vi "Mock Circulation Loop met sub-Vi - AANGEPAST VOOR CHARLOTTE.vi"() -> ()   [LabVIEW 2024]
uses:
  <vilib>/DAQmx/write.llb/DAQmx Write (Analog DBL 1Chan 1Samp).vi
  <vilib>/DAQmx/read.llb/DAQmx Read (Analog 1D DBL NChan 1Samp).vi
  <vilib>/DAQmx/write.llb/DAQmx Write (Digital 1D Bool NChan 1Samp 1Line).vi
  <vilib>/DAQmx/create/channels.llb/DAQmx Create Channel (DO-Digital Output).vi
  <vilib>/DAQmx/miscellaneous.llb/DAQmx Fill In Error Info.vi
  <vilib>/DAQmx/create/channels.llb/DAQmx Create Channel (AI-Voltage-Basic).vi
  <vilib>/DAQmx/create/channels.llb/DAQmx Create Channel (AO-Voltage-Basic).vi
  <vilib>/Utility/file.llb/Write Delimited Spreadsheet (string).vi
  <vilib>/Utility/file.llb/Write Delimited Spreadsheet (DBL).vi
panel:
  in  "Set pressure Hybrid Heart (Bar)":dbl
  in  "Analog output pressure regulator":tag="Dev1/ao0"
  out "Actual Press. from Regulator (Bar)":dbl=0.5073311185231432
  out "Flow sensors":cluster{dbl[], dbl[]}[](graph)=[{[0.014721000000463391], [-6.750071131370961, -6.750071131370961, -6.750071131370961, -6.750071131370961, -6.750071131370961, -6.750071131370961, -6.750071131370961, -6.750071131370961, -6.750071131370961, -6.750071131370961, -6.750071131370961, -6.750071131370961, -6.750071131370961, -6.750071131370961, -6.750071131370961, -6.750071131370961, -6.755156296628295, -6.755156296628295, -6.750071131370961, -6.750071131370961, -6.750071131370961, -6.750071131370961, -6.750071131370961, -6.750071131370961, -6.750071131370961, -6.750071131370961, -6.750071131370961, -6.755156296628295, -6.750071131370961, -6.750071131370961, -6.750071131370961, -6.750071131370961, -6.750071131370961, -6.750071131370961, -6.750071131370961, -6.750071131370961, -6.750071131370961, -6.750071131370961, -6.750071131370961, -6.750071131370961, -6.750071131370961, -6.750071131370961, -6.750071131370961, -6.750071131370961, -6.750071131370961, -6.750071131370961, -6.750071131370961, -6.750071131370961, -6.750071131370961, -6.750071131370961, -6.750071131370961, -6.750071131370961, -6.750071131370961, -6.750071131370961, -6.750071131370961, -6.750071131370961, -6.750071131370961, -6.750071131370961, -6.750071131370961, -6.750071131370961, -6.750071131370961, -6.750071131370961, -6.750071131370961, -6.750071131370961, -6.750071131370961, -6.750071131370961, -6.750071131370961, -6.750071131370961, -6.750071131370961, -6.750071131370961, -6.755156296628295, -6.750071131370961, -6.750071131370961, -6.750071131370961, -6.750071131370961, -6.750071131370961, -6.755156296628295, -6.750071131370961, -6.750071131370961, -6.750071131370961, -6.750071131370961, -6.750071131370961, -6.750071131370961, -6.750071131370961, -6.750071131370961, -6.750071131370961, -6.750071131370961, -6.750071131370961, -6.750071131370961, -6.750071131370961, -6.750071131370961, -6.750071131370961, -6.750071131370961, -6.755156296628295, -6.744985966113629, -6.750071131370961, -6.750071131370961, -6.750071131370961, -6.750071131370961, -6.750071131370961, -6.750071131370961, -6.750071131370961, -6.750071131370961, -6.750071131370961, -6.750071131370961, -6.750071131370961, -6.750071131370961, -6.750071131370961, -6.755156296628295, -6.750071131370961, -6.750071131370961, -6.750071131370961, -6.750071131370961, -6.755156296628295, -6.750071131370961, -6.750071131370961, -6.750071131370961, -6.750071131370961, -6.750071131370961, -6.750071131370961, -6.755156296628295, -6.750071131370961, -6.750071131370961, -6.750071131370961, -6.750071131370961, -6.750071131370961, -6.750071131370961, -6.750071131370961, -6.750071131370961, -6.750071131370961, -6.750071131370961, -6.755156296628295, -6.750071131370961, -6.750071131370961, -6.750071131370961, -6.750071131370961, -6.750071131370961, -6.750071131370961, -6.750071131370961, -6.750071131370961, -6.750071131370961, -6.750071131370961, -6.750071131370961, -6.750071131370961, -6.750071131370961, -6.750071131370961, -6.755156296628295, -6.750071131370961, -6.750071131370961, -6.750071131370961, -6.750071131370961, -6.750071131370961, -6.750071131370961, -6.750071131370961, -6.750071131370961, -6.750071131370961, -6.750071131370961, -6.750071131370961, -6.750071131370961, -6.750071131370961, -6.750071131370961, -6.750071131370961, -6.750071131370961, -6.750071131370961, -6.750071131370961, -6.750071131370961, -6.750071131370961, -6.750071131370961, -6.744985966113629, -6.750071131370961, -6.750071131370961, -6.750071131370961, -6.750071131370961, -6.750071131370961, -6.750071131370961, -6.750071131370961, -6.750071131370961, -6.750071131370961, -6.750071131370961, -6.750071131370961, -6.750071131370961, -6.750071131370961, -6.750071131370961, -6.750071131370961, -6.750071131370961, -6.750071131370961, -6.750071131370961, -6.750071131370961, -6.750071131370961, -6.755156296628295, -6.755156296628295, -6.750071131370961, -6.750071131370961, -6.750071131370961, -6.750071131370961, -6.750071131370961, -6.750071131370961, -6.750071131370961, -6.744985966113629, -6.750071131370961, -6.750071131370961, -6.750071131370961, -6.750071131370961, -6.750071131370961, -6.750071131370961, -6.750071131370961, -6.750071131370961, -6.750071131370961, -6.750071131370961, -6.750071131370961, -6.750071131370961, -6.750071131370961, -6.750071131370961, -6.755156296628295, -6.750071131370961, -6.750071131370961, -6.750071131370961, -6.750071131370961, -6.750071131370961, -6.755156296628295, -6.750071131370961, -6.750071131370961, -6.750071131370961, -6.750071131370961, -6.750071131370961, -6.750071131370961, -6.750071131370961, -6.750071131370961, -6.750071131370961, -6.750071131370961, -6.750071131370961, -6.750071131370961, -6.750071131370961, -6.750071131370961, -6.750071131370961, -6.750071131370961, -6.750071131370961, -6.750071131370961, -6.750071131370961, -6.750071131370961, -6.750071131370961, -6.750071131370961, -6.750071131370961, -6.750071131370961, -6.750071131370961, -6.750071131370961, -6.750071131370961, -6.750071131370961, -6.750071131370961, -6.750071131370961, -6.750071131370961, -6.750071131370961, -6.750071131370961, -6.755156296628295, -6.750071131370961, -6.750071131370961, -6.750071131370961, -6.755156296628295, -6.750071131370961, -6.750071131370961, -6.750071131370961, -6.750071131370961, -6.750071131370961, -6.750071131370961, -6.755156296628295, -6.750071131370961, -6.750071131370961, -6.750071131370961, -6.750071131370961, -6.750071131370961, -6.750071131370961, -6.750071131370961, -6.750071131370961, -6.750071131370961, -6.750071131370961, -6.750071131370961, -6.750071131370961, -6.750071131370961, -6.750071131370961, -6.750071131370961, -6.750071131370961, -6.750071131370961, -6.750071131370961, -6.750071131370961, -6.750071131370961, -6.750071131370961, -6.750071131370961, -6.750071131370961, -6.750071131370961, -6.750071131370961, -6.755156296628295, -6.750071131370961, -6.750071131370961, -6.750071131370961, -6.750071131370961, -6.750071131370961, -6.750071131370961, -6.750071131370961, -6.750071131370961, -6.755156296628295, -6.750071131370961, -6.750071131370961, -6.750071131370961, -6.750071131370961, -6.755156296628295, -6.750071131370961, -6.755156296628295, -6.750071131370961, -6.750071131370961, -6.750071131370961, -6.750071131370961, -6.750071131370961, -6.750071131370961, -6.750071131370961, -6.750071131370961, -6.750071131370961, -6.750071131370961, -6.750071131370961, -6.750071131370961, -6.750071131370961, -6.750071131370961, -6.750071131370961, -6.750071131370961, -6.750071131370961, -6.750071131370961, -6.750071131370961, -6.750071131370961, -6.750071131370961, -6.750071131370961, -6.750071131370961, -6.750071131370961, -6.750071131370961, -6.750071131370961, -6.750071131370961, -6.750071131370961, -6.750071131370961, -6.750071131370961, -6.750071131370961, -6.750071131370961, -6.750071131370961, -6.750071131370961, -6.750071131370961, -6.750071131370961, -6.750071131370961, -6.750071131370961, -6.750071131370961, -6.755156296628295, -6.750071131370961, -6.750071131370961, -6.750071131370961, -6.750071131370961, -6.750071131370961, -6.750071131370961, -6.750071131370961, -6.750071131370961, -6.750071131370961, -6.755156296628295, -6.750071131370961, -6.750071131370961, -6.750071131370961, -6.750071131370961, -6.750071131370961, -6.750071131370961, -6.750071131370961, -6.750071131370961, -6.750071131370961, -6.750071131370961, -6.750071131370961, -6.750071131370961, -6.750071131370961, -6.750071131370961, -6.750071131370961, -6.750071131370961, -6.750071131370961, -6.750071131370961, -6.750071131370961, -6.750071131370961, -6.750071131370961, -6.750071131370961, -6.750071131370961, -6.750071131370961, -6.750071131370961, -6.750071131370961, -6.750071131370961, -6.750071131370961, -6.750071131370961, -6.750071131370961, -6.744985966113629, -6.750071131370961, -6.750071131370961, -6.750071131370961, -6.750071131370961, -6.750071131370961, -6.750071131370961, -6.750071131370961, -6.755156296628295, -6.750071131370961, -6.750071131370961, -6.750071131370961, -6.750071131370961, -6.750071131370961, -6.750071131370961, -6.750071131370961, -6.755156296628295, -6.750071131370961]}, ...(2 in all)]
  in  "Seconds per data point":dbl
  out "Pressure sensors":cluster{dbl[], dbl[]}[](graph)=[{[0.014721000000463391], [-2.2408081975299865, -2.2408081975299865, -2.4339157389476895, -2.2408081975299865, -1.8545931146945804, -2.4339157389476895, -2.2408081975299865, -2.2408081975299865, -2.2408081975299865, -2.2408081975299865, -2.4339157389476895, -2.4339157389476895, -2.4339157389476895, -2.4339157389476895, -2.4339157389476895, -2.2408081975299865, -2.2408081975299865, -2.2408081975299865, -2.4339157389476895, -2.2408081975299865, -2.4339157389476895, -2.2408081975299865, -2.4339157389476895, -2.2408081975299865, -2.2408081975299865, -2.2408081975299865, -2.2408081975299865, -2.2408081975299865, -2.4339157389476895, -2.2408081975299865, -2.4339157389476895, -2.2408081975299865, -2.4339157389476895, -2.4339157389476895, -2.4339157389476895, -2.4339157389476895, -2.4339157389476895, -2.2408081975299865, -2.2408081975299865, -2.2408081975299865, -2.4339157389476895, -2.2408081975299865, -2.4339157389476895, -2.4339157389476895, -2.4339157389476895, -2.2408081975299865, -2.2408081975299865, -2.2408081975299865, -2.4339157389476895, -2.2408081975299865, -2.4339157389476895, -2.4339157389476895, -2.2408081975299865, -2.2408081975299865, -2.4339157389476895, -2.4339157389476895, -2.2408081975299865, -2.2408081975299865, -2.2408081975299865, -2.4339157389476895, -2.4339157389476895, -2.2408081975299865, -2.4339157389476895, -2.4339157389476895, -2.4339157389476895, -2.4339157389476895, -2.4339157389476895, -2.4339157389476895, -2.2408081975299865, -2.2408081975299865, -2.2408081975299865, -2.4339157389476895, -2.2408081975299865, -2.4339157389476895, -2.2408081975299865, -2.2408081975299865, -2.4339157389476895, -2.4339157389476895, -2.4339157389476895, -2.4339157389476895, -2.4339157389476895, -2.4339157389476895, -2.4339157389476895, -2.4339157389476895, -2.4339157389476895, -2.4339157389476895, -2.4339157389476895, -2.2408081975299865, -2.4339157389476895, -2.4339157389476895, -2.2408081975299865, -2.4339157389476895, -2.4339157389476895, -2.2408081975299865, -2.4339157389476895, -2.4339157389476895, -2.4339157389476895, -2.2408081975299865, -2.4339157389476895, -2.4339157389476895, -2.4339157389476895, -2.2408081975299865, -2.4339157389476895, -2.4339157389476895, -2.2408081975299865, -2.2408081975299865, -2.4339157389476895, -2.4339157389476895, -2.2408081975299865, -2.4339157389476895, -2.4339157389476895, -2.0477006561122835, -2.4339157389476895, -2.2408081975299865, -2.4339157389476895, -2.2408081975299865, -2.2408081975299865, -2.4339157389476895, -2.0477006561122835, -2.2408081975299865, -2.2408081975299865, -2.4339157389476895, -2.2408081975299865, -2.4339157389476895, -2.4339157389476895, -2.4339157389476895, -2.4339157389476895, -2.4339157389476895, -2.2408081975299865, -2.0477006561122835, -2.4339157389476895, -2.4339157389476895, -2.4339157389476895, -2.2408081975299865, -2.4339157389476895, -2.4339157389476895, -2.4339157389476895, -2.4339157389476895, -2.2408081975299865, -2.4339157389476895, -2.4339157389476895, -2.4339157389476895, -2.2408081975299865, -2.4339157389476895, -2.4339157389476895, -2.4339157389476895, -2.4339157389476895, -2.4339157389476895, -2.2408081975299865, -2.4339157389476895, -2.4339157389476895, -1.8545931146945804, -2.2408081975299865, -2.4339157389476895, -2.2408081975299865, -2.2408081975299865, -2.4339157389476895, -2.2408081975299865, -2.4339157389476895, -2.0477006561122835, -2.4339157389476895, -2.2408081975299865, -2.0477006561122835, -2.4339157389476895, -2.4339157389476895, -2.2408081975299865, -2.2408081975299865, -2.4339157389476895, -2.2408081975299865, -2.4339157389476895, -2.2408081975299865, -2.4339157389476895, -2.2408081975299865, -2.2408081975299865, -2.4339157389476895, -2.4339157389476895, -2.4339157389476895, -2.0477006561122835, -2.2408081975299865, -2.4339157389476895, -2.2408081975299865, -2.4339157389476895, -2.2408081975299865, -2.4339157389476895, -2.4339157389476895, -2.4339157389476895, -2.4339157389476895, -2.2408081975299865, -2.4339157389476895, -2.4339157389476895, -2.2408081975299865, -2.2408081975299865, -2.4339157389476895, -2.4339157389476895, -2.2408081975299865, -2.4339157389476895, -2.4339157389476895, -2.2408081975299865, -2.2408081975299865, -2.4339157389476895, -2.4339157389476895, -2.2408081975299865, -2.2408081975299865, -2.2408081975299865, -2.2408081975299865, -2.2408081975299865, -2.4339157389476895, -2.4339157389476895, -2.4339157389476895, -2.2408081975299865, -2.4339157389476895, -2.2408081975299865, -2.4339157389476895, -2.6270232803653926, -2.4339157389476895, -2.2408081975299865, -2.2408081975299865, -2.2408081975299865, -2.4339157389476895, -2.4339157389476895, -2.2408081975299865, -2.4339157389476895, -2.4339157389476895, -2.2408081975299865, -2.4339157389476895, -2.4339157389476895, -2.4339157389476895, -2.2408081975299865, -2.4339157389476895, -1.8545931146945804, -2.4339157389476895, -2.4339157389476895, -2.4339157389476895, -2.4339157389476895, -2.4339157389476895, -2.0477006561122835, -2.4339157389476895, -2.4339157389476895, -2.2408081975299865, -2.4339157389476895, -2.2408081975299865, -2.4339157389476895, -2.4339157389476895, -2.4339157389476895, -2.2408081975299865, -2.2408081975299865, -1.8545931146945804, -2.4339157389476895, -2.4339157389476895, -2.2408081975299865, -2.4339157389476895, -2.4339157389476895, -2.4339157389476895, -2.4339157389476895, -2.4339157389476895, -2.4339157389476895, -2.4339157389476895, -2.2408081975299865, -2.2408081975299865, -2.4339157389476895, -2.4339157389476895, -2.4339157389476895, -2.2408081975299865, -2.4339157389476895, -2.4339157389476895, -2.4339157389476895, -2.4339157389476895, -2.4339157389476895, -2.4339157389476895, -2.4339157389476895, -2.4339157389476895, -2.4339157389476895, -2.4339157389476895, -2.2408081975299865, -2.4339157389476895, -2.4339157389476895, -2.2408081975299865, -2.4339157389476895, -2.2408081975299865, -2.2408081975299865, -2.4339157389476895, -2.4339157389476895, -2.2408081975299865, -2.4339157389476895, -2.4339157389476895, -2.4339157389476895, -2.2408081975299865, -2.4339157389476895, -2.2408081975299865, -2.4339157389476895, -2.2408081975299865, -2.4339157389476895, -2.4339157389476895, -2.2408081975299865, -2.2408081975299865, -2.4339157389476895, -2.4339157389476895, -1.8545931146945804, -2.4339157389476895, -2.2408081975299865, -2.2408081975299865, -2.4339157389476895, -2.4339157389476895, -2.2408081975299865, -2.4339157389476895, -2.2408081975299865, -2.4339157389476895, -2.2408081975299865, -2.4339157389476895, -2.2408081975299865, -2.2408081975299865, -2.2408081975299865, -2.2408081975299865, -2.2408081975299865, -2.2408081975299865, -2.4339157389476895, -2.2408081975299865, -2.4339157389476895, -2.4339157389476895, -2.4339157389476895, -2.2408081975299865, -2.4339157389476895, -2.4339157389476895, -2.4339157389476895, -2.2408081975299865, -2.2408081975299865, -2.2408081975299865, -2.4339157389476895, -2.2408081975299865, -2.4339157389476895, -2.4339157389476895, -2.4339157389476895, -2.2408081975299865, -2.4339157389476895, -2.4339157389476895, -2.2408081975299865, -2.4339157389476895, -2.4339157389476895, -2.4339157389476895, -2.2408081975299865, -2.4339157389476895, -2.4339157389476895, -2.2408081975299865, -2.4339157389476895, -2.0477006561122835, -2.4339157389476895, -2.4339157389476895, -2.4339157389476895, -2.2408081975299865, -2.4339157389476895, -2.4339157389476895, -2.2408081975299865, -2.4339157389476895, -2.4339157389476895, -2.2408081975299865, -2.4339157389476895, -2.2408081975299865, -2.4339157389476895, -2.4339157389476895, -2.4339157389476895, -2.2408081975299865, -2.4339157389476895, -2.4339157389476895, -2.4339157389476895, -2.2408081975299865, -2.4339157389476895, -2.4339157389476895, -2.4339157389476895, -2.2408081975299865, -2.4339157389476895, -2.2408081975299865, -2.4339157389476895, -2.4339157389476895, -2.4339157389476895, -2.2408081975299865, -1.8545931146945804, -2.4339157389476895, -2.2408081975299865, -2.4339157389476895, -2.4339157389476895, -2.2408081975299865, -2.2408081975299865, -2.4339157389476895, -2.2408081975299865, -2.4339157389476895, -2.4339157389476895, -2.2408081975299865, -2.4339157389476895, -2.2408081975299865, -2.2408081975299865, -2.4339157389476895, -2.2408081975299865, -2.2408081975299865, -2.2408081975299865, -2.4339157389476895, -2.4339157389476895, -2.4339157389476895, -2.4339157389476895, -2.2408081975299865, -2.4339157389476895, -2.2408081975299865, -2.4339157389476895, -2.4339157389476895, -2.2408081975299865, -2.2408081975299865]}, ...(2 in all)]
  out "Elapsed time":dbl=0.014721000000463391
  in  "Input port all sensors":tag="Dev1/ai3:7"
  in  "Start/Stop solenoid valves":bool
  in  "Closed time (ms)":dbl=700.0
  in  "Open time (ms)":dbl=300.0
  in  "STOP":bool
  in  "line grouping":i32(ring) items=["one channel for each line", "one channel for all lines"]
  in  "Port input Solenoid valve":tag="Dev1/port0/line0:1"
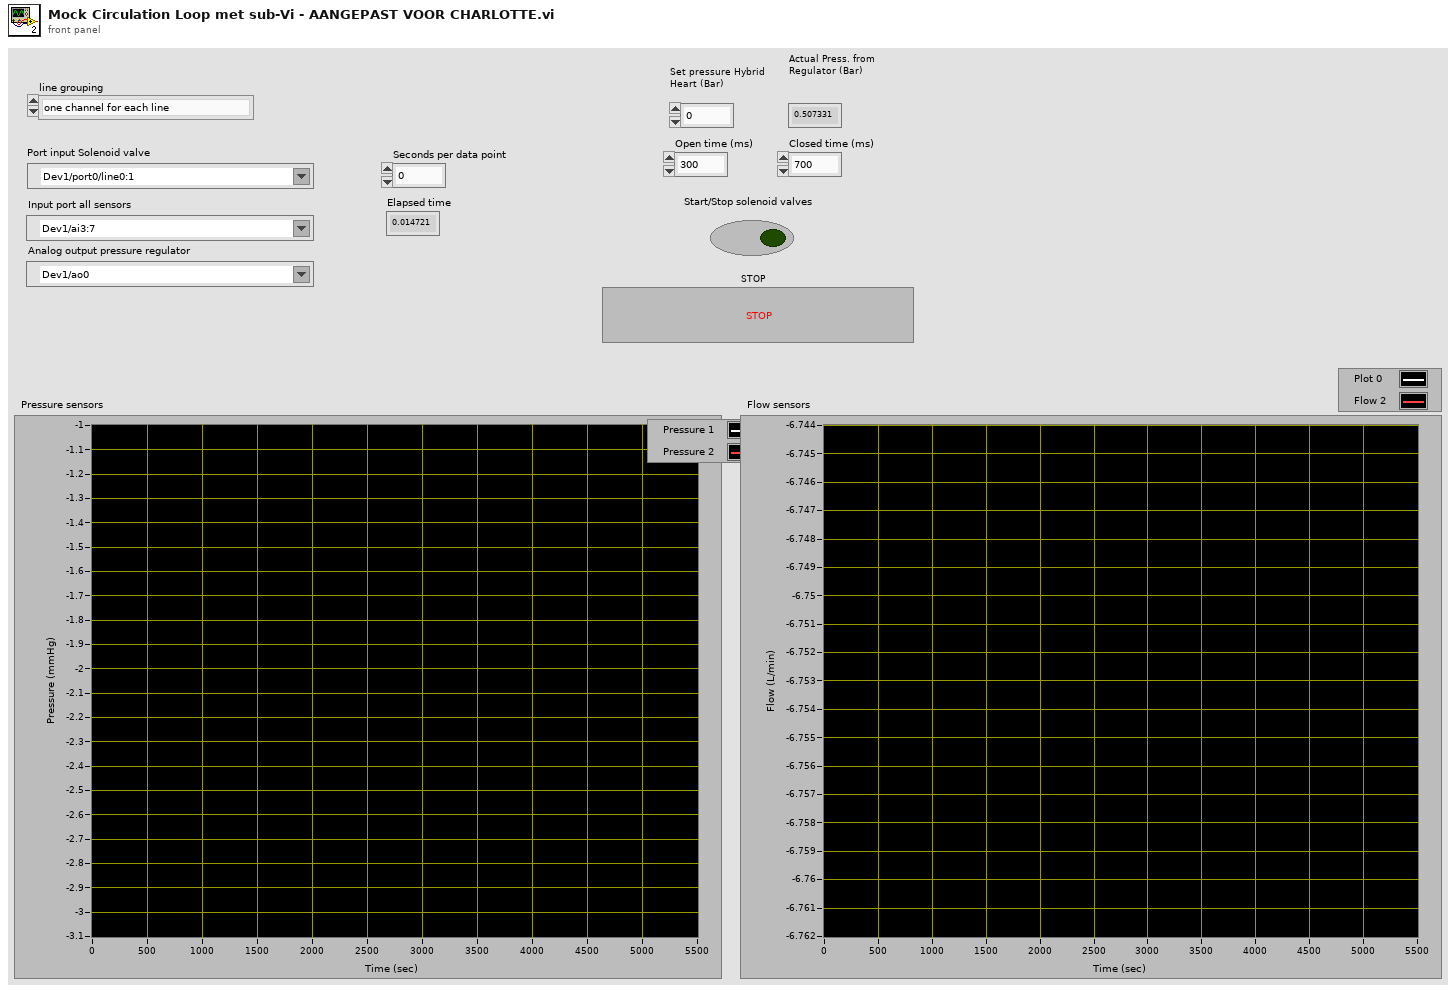
[diagram p1: front panel]
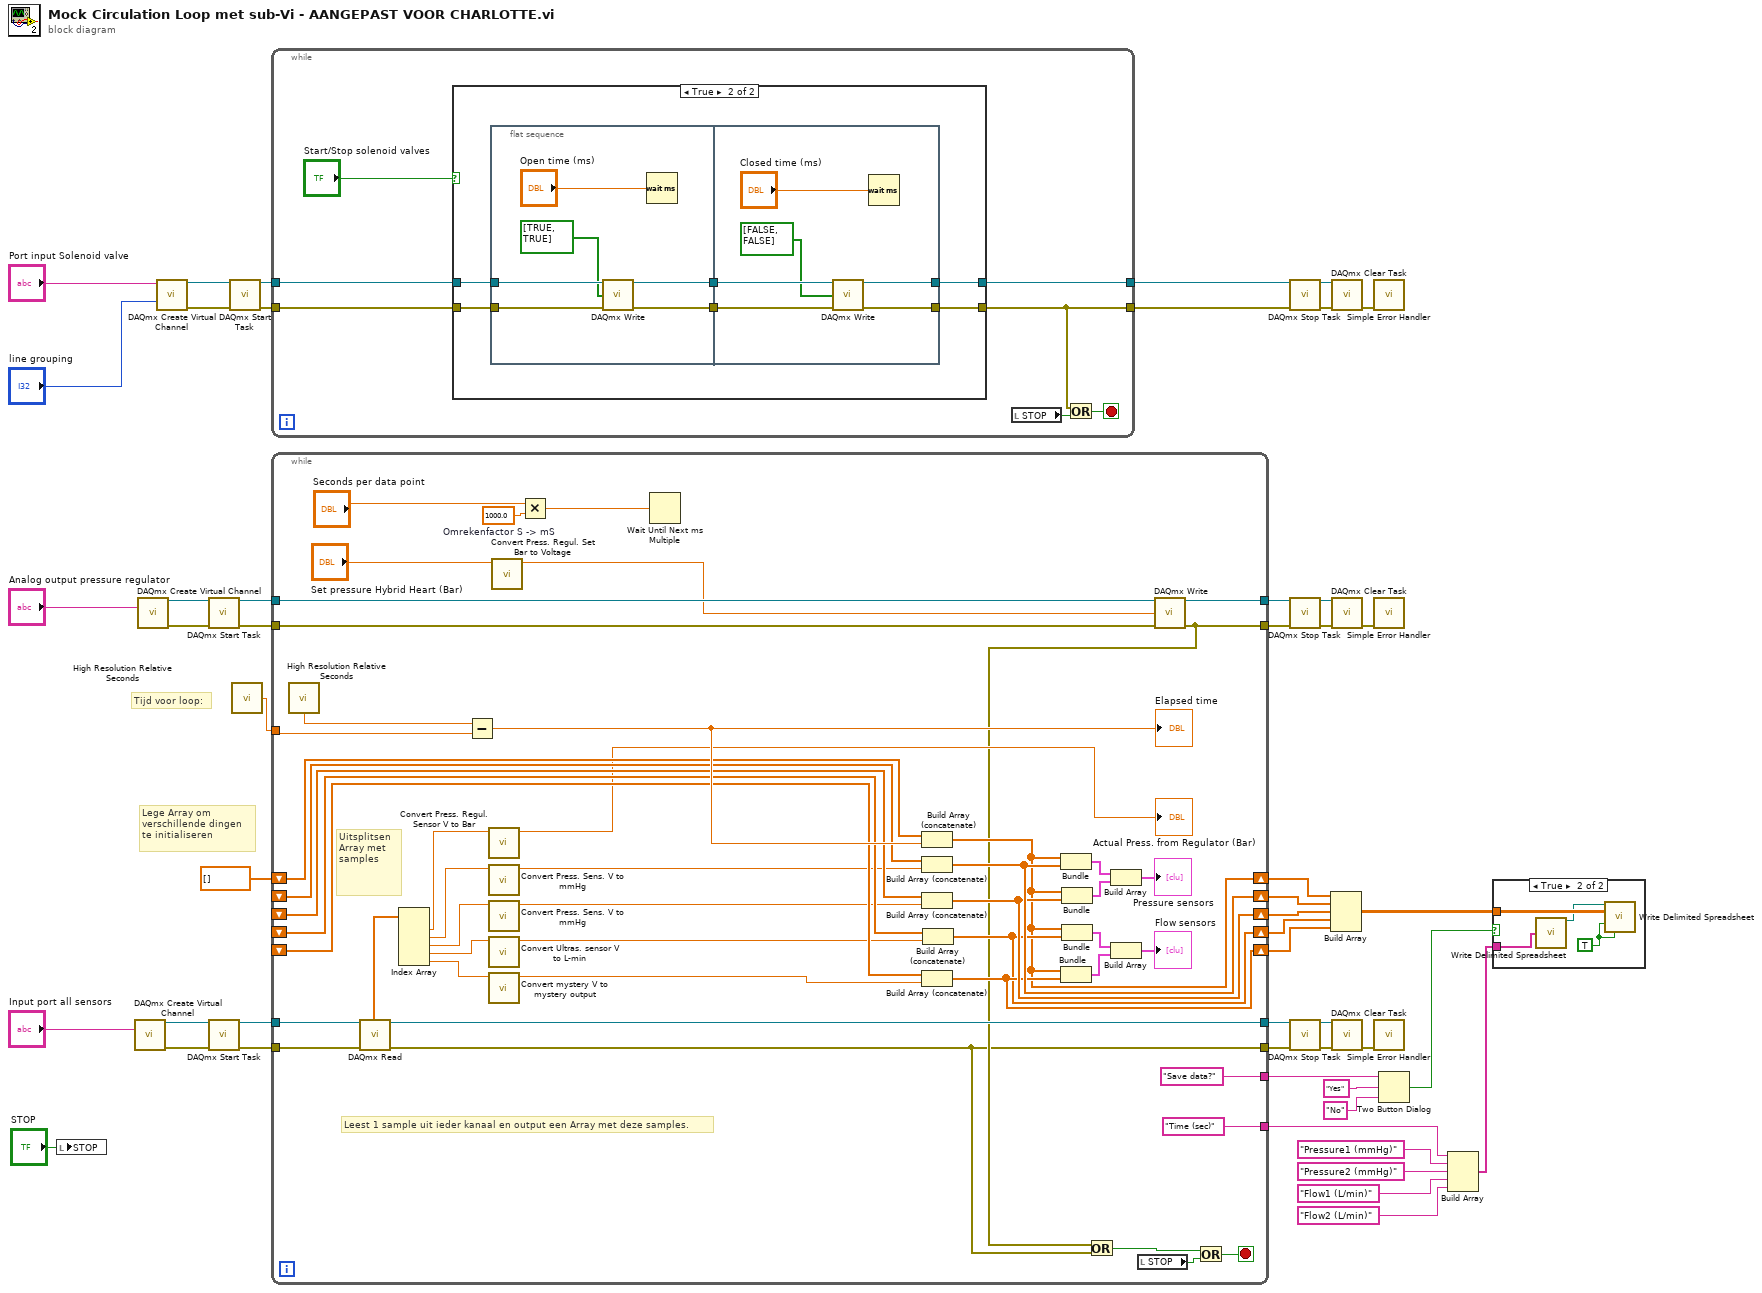
[diagram p0: block diagram]
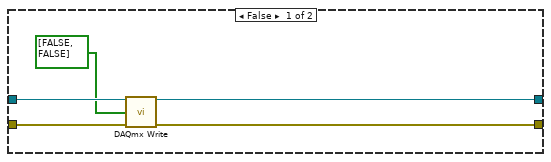
[diagram p3: hidden frame]
diagram:
  # "Tijd voor loop:"
  # "Lege Array om\nverschillende dingen \nte initialiseren"
  n1 = local write "STOP"("STOP") -> ()
  n2 = call-poly <vilib>:"DAQmx Create Virtual Channel.vi"("physical channels"="Input port all sensors") -> ("task out"=w36:refnum<k21>, "error out"=w35:errorcluster)  [unwired: 13 in]
  n3 = call-poly <vilib>:"DAQmx Create Virtual Channel.vi"("physical channels"="Analog output pressure regulator") -> ("task out"=w27:refnum<k21>, "error out"=w26:errorcluster)  [unwired: 13 in]
  n4 = call-poly <vilib>:"DAQmx Create Virtual Channel.vi"("lines"="Port input Solenoid valve", "line grouping"="line grouping") -> ("task out"=w48:refnum<k21>, "error out"=w49:errorcluster)  [unwired: 12 in]
  n5 = call <vilib>:"DAQmx Start Task.vi"("task/channels in"=w27, "error in"=w26) -> ("task out"=w23:refnum<k21>, "error out"=w24:errorcluster)  [unwired: 12 in]
  n6 = call <vilib>:"DAQmx Start Task.vi"("task/channels in"=w36, "error in"=w35) -> ("task out"=w34:refnum<k21>, "error out"=w33:errorcluster)  [unwired: 12 in]
  n7 = call <vilib>:"DAQmx Start Task.vi"("task/channels in"=w48, "error in"=w49) -> ("task out"=w46:refnum<k21>, "error out"=w45:errorcluster)  [unwired: 12 in]
  n8 = call <vilib>:"High Resolution Relative Seconds.vi"() -> ("relative seconds"=w38:dbl)
  n9 = while {
    tunnel: w46 -> [w56]
    tunnel: w45 -> [w55]
    tunnel: [w52] -> w43
    tunnel: [w54] -> w42
    stop <- w53 stop-if-true
    n10 = case shown="True" "Start/Stop solenoid valves" {
      tunnel: w56 -> [w62 w66]
      tunnel: w55 -> [w61 w65]
      tunnel: [w59 w64] -> w52
      tunnel: [w58 w63] -> w54
      frame False {
        n11 = call-poly <vilib>:"DAQmx Write.vi"("task/channels in"=w62, "data"=bool[] [FALSE, FALSE], "error in"=w61) -> ("task out"=w58:refnum<k21>, "error out"=w59:errorcluster)  [unwired: 10 in, 1 out]
      }
      frame True {
        n12 = flat-sequence {
          tunnel: w66 -> [w74]
          tunnel: w65 -> [w73]
          tunnel: [w71] -> w68
          tunnel: [w70] -> w67
          tunnel: w68 -> [w79]
          tunnel: w67 -> [w78]
          tunnel: [w77] -> w63
          tunnel: [w76] -> w64
          frame #0 {
            n13 = call-poly <vilib>:"DAQmx Write.vi"("task/channels in"=w74, "data"=bool[] [TRUE, TRUE], "error in"=w73) -> ("task out"=w71:refnum<k21>, "error out"=w70:errorcluster)  [unwired: 10 in, 1 out]
            n14 = Wait (ms)(milliseconds to wait="Open time (ms)") -> ()  [unwired: 1 out]
          }
          frame #1 {
            n15 = call-poly <vilib>:"DAQmx Write.vi"("task/channels in"=w79, "data"=bool[] [FALSE, FALSE], "error in"=w78) -> ("task out"=w77:refnum<k21>, "error out"=w76:errorcluster)  [unwired: 10 in, 1 out]
            n16 = Wait (ms)(milliseconds to wait="Closed time (ms)") -> ()  [unwired: 1 out]
          }
        }
      }
    }
    n17 = local read "STOP"() -> (w51:bool)
    n18 = Or(x=w52, y=w51) -> (x .or. y?=w53:bool)
  }
  n19 = while {
    tunnel: w34 -> [w128]
    tunnel: w33 -> [w127]
    tunnel: w38 -> [w122]
    shift-right: [w106] -> w17
    shift-left: dbl[] [] -> [w120]
    shift-right: [w116] -> w16
    shift-left: _ -> [w118]
    shift-right: [w115] -> w15
    shift-left: _ -> [w117]
    tunnel: [w111] -> w32
    tunnel: [w82] -> w31
    shift-right: [w107] -> w14
    shift-left: _ -> [w110]
    shift-right: [w108] -> w13
    shift-left: _ -> [w109]
    tunnel: w24 -> [w81]
    tunnel: w23 -> [w102]
    tunnel: [w83] -> w19
    tunnel: [w101] -> w18
    tunnel: ["Time (sec)"] -> w6
    tunnel: ["Save data?" ("message")] -> w2
    stop <- w93 stop-if-true
    w124 = 1000.0  # Omrekenfactor S -> mS
    # "Leest 1 sample uit ieder kanaal en output een Array met deze samples."
    # "Uitsplitsen Array met \nsamples"
    n20 = call <vilib>:"High Resolution Relative Seconds.vi"() -> ("relative seconds"=w123:dbl)
    n21 = call-poly <vilib>:"DAQmx Read.vi"("task/channels in"=w128, "error in"=w127) -> ("task out"=w111:refnum<k21>, "data"=w119:dbl[], "error out"=w82:errorcluster)  [unwired: 11 in]
    n22 = Index Array(array=w119) -> (element #1=w100:dbl, element #2=w86:dbl, element #3=w85:dbl, element #4=w88:dbl, element #5=w87:dbl)  [unwired: 5 in]
    n23 = Subtract(x=w123, y=w122) -> (x-y=w121:dbl)
    "Elapsed time" <- w121
    n24 = call "Convert Press. Regul. Sensor V to Bar.vi"("V. Regulator Press. Sensor"=w100) -> ("Press. at Regulator (Bar)"=→"Actual Press. from Regulator (Bar)":dbl)  [unwired: 10 in]
    n25 = call "Convert Press. Sens. V to mmHg.vi"("Waveform"=w86) -> ("Numeric"=w89:dbl)  [unwired: 10 in]
    n26 = call "Convert Press. Sens. V to mmHg.vi"("Waveform"=w85) -> ("Numeric"=w84:dbl)  [unwired: 10 in]
    n27 = call "Convert Ultras. sensor V to L-min.vi"("Waveform"=w88) -> ("Numeric"=w91:dbl)  [unwired: 10 in]
    n28 = call "Convert mystery V to mystery output.vi"("Waveform"=w87) -> ("Numeric"=w90:dbl)  [unwired: 10 in]
    n29 = call "Convert Press. Regul. Set Bar to Voltage.vi"("Set pressure Hybrid Heart (Bar)"="Set pressure Hybrid Heart (Bar)") -> ("Numeric"=w97:dbl)  [unwired: 10 in]
    n30 = Multiply(x="Seconds per data point", y=w124) -> (x*y=w126:dbl)
    n31 = Wait Until Next ms Multiple(millisecond multiple=w126) -> ()  [unwired: 1 out]
    n32 = Build Array (concatenate)(w120, w121) -> (w106:dbl[])
    n33 = Build Array (concatenate)(w118, w89) -> (w116:dbl[])
    n34 = Build Array (concatenate)(w117, w84) -> (w115:dbl[])
    n35 = Build Array (concatenate)(w109, w90) -> (w108:dbl[])
    n36 = Build Array (concatenate)(w110, w91) -> (w107:dbl[])
    n37 = Bundle(w106, w116) -> (w114:cluster{dbl[], dbl[]})  [unwired: 1 in]
    n38 = Bundle(w106, w108) -> (w104:cluster{dbl[], dbl[]})  [unwired: 1 in]
    n39 = Bundle(w106, w115) -> (w113:cluster{dbl[], dbl[]})  [unwired: 1 in]
    n40 = Bundle(w106, w107) -> (w105:cluster{dbl[], dbl[]})  [unwired: 1 in]
    n41 = Build Array(w114, w113) -> (→"Pressure sensors":cluster{dbl[], dbl[]}[])
    n42 = Build Array(w105, w104) -> (→"Flow sensors":cluster{dbl[], dbl[]}[])
    n43 = local read "STOP"() -> (w92:bool)
    n44 = call-poly <vilib>:"DAQmx Write.vi"("task/channels in"=w102, "data"=w97, "error in"=w81) -> ("task out"=w101:refnum<k21>, "error out"=w83:errorcluster)  [unwired: 10 in, 1 out]
    n45 = Or(x=w83, y=w82) -> (x .or. y?=w94:bool)
    n46 = Or(x=w94, y=w92) -> (x .or. y?=w93:bool)
  }
  n47 = call <vilib>:"DAQmx Stop Task.vi"("task/channels in"=w42, "error in"=w43) -> ("task out"=w41:refnum<k21>, "error out"=w40:errorcluster)  [unwired: 12 in]
  n48 = call <vilib>:"DAQmx Stop Task.vi"("task/channels in"=w18, "error in"=w19) -> ("task out"=w21:refnum<k21>, "error out"=w22:errorcluster)  [unwired: 12 in]
  n49 = call <vilib>:"DAQmx Stop Task.vi"("task/channels in"=w32, "error in"=w31) -> ("task out"=w29:refnum<k21>, "error out"=w30:errorcluster)  [unwired: 12 in]
  n50 = Build Array(w17, w16, w15, w14, w13) -> (w12:dbl[][])
  n51 = call <vilib>:"DAQmx Clear Task.vi"("task in"=w41, "error in"=w40) -> ("error out"=w44:errorcluster)  [unwired: 13 in]
  n52 = call <vilib>:"DAQmx Clear Task.vi"("task in"=w21, "error in"=w22) -> ("error out"=w20:errorcluster)  [unwired: 13 in]
  n53 = call <vilib>:"DAQmx Clear Task.vi"("task in"=w29, "error in"=w30) -> ("error out"=w28:errorcluster)  [unwired: 13 in]
  n54 = call <vilib>:"Simple Error Handler.vi"("error in (no error)"=w44) -> ()  [unwired: 4 in, 5 out]
  n55 = call <vilib>:"Simple Error Handler.vi"("error in (no error)"=w20) -> ()  [unwired: 4 in, 5 out]
  n56 = call <vilib>:"Simple Error Handler.vi"("error in (no error)"=w28) -> ()  [unwired: 4 in, 5 out]
  n57 = Two Button Dialog(message=w2, 1:"No" ("F button name (\"Cancel\")"), 2:"Yes" ("T button name (\"OK\")")) -> (T button?=w5:bool)
  n58 = Build Array(w6, "Pressure1 (mmHg)", "Pressure2 (mmHg)", "Flow1 (L/min)", "Flow2 (L/min)") -> (w7:string[])
  n59 = case shown="True" w5 {
    tunnel: w12 -> [_ w132]
    tunnel: w7 -> [_ w131]
    frame False {
    }
    frame True {
      w129 = TRUE ("transpose? (no:F)")
      n60 = call-poly <vilib>:"Write Delimited Spreadsheet.vi"("1D data"=w131) -> ("new file path (Not A Path if cancelled)"=w130:path)  [unwired: 13 in, 1 out]
      n61 = call-poly <vilib>:"Write Delimited Spreadsheet.vi"("file path (dialog if empty)"=w130, "2D data"=w132, "append to file? (new file:F)"=w129, "transpose? (no:F)"=w129) -> ()  [unwired: 10 in, 2 out]
    }
  }
